vi "Write Log.vi"(7 "Prepend timestamp":bool, 10 "Log entry":string, 11 "SolutionBuilder in":refnum<class "SolutionBuilder.lvclass">) -> (3 "SolutionBuilder out":refnum<class "SolutionBuilder.lvclass">)   [LabVIEW 2019, in "SolutionBuilder.lvlib" / "SolutionBuilder.lvclass"]
uses:
  SolutionBuilder.lvclass
  SolutionBuilder.lvclass/SolutionBuilder.ctl
  SolutionBuilder.lvlib
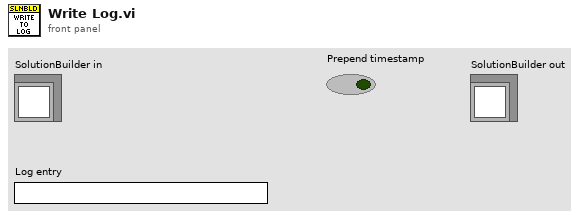
[diagram p1: front panel]
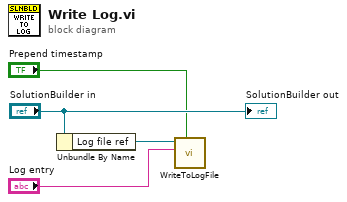
[diagram p0: block diagram]
diagram:
  n1 = Unbundle By Name("SolutionBuilder in") -> ("Log file ref"=w3:refnum<file>)
  n2 = call "WriteToLogFile.vi"("Prepend timestamp"="Prepend timestamp", "Log entry"="Log entry", "Byte Stream File in"=w3) -> ()  [unwired: 7 in, 2 out]
  "SolutionBuilder out" <- "SolutionBuilder in"
